vi "Bartender打印子vi.vi"   [LabVIEW 2024]
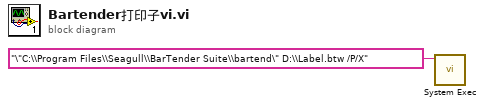
[diagram p0: block diagram]
diagram:
  n1 = call <vilib>:"System Exec.vi"("command line"="\"C:\\Program Files\\Seagull\\BarTender Suite\\bartend\" D:\\Label.btw /P/X") -> ()  [unwired: 7 in, 4 out]
